vi "VIH Utility - VISRV - Get Datatype Terminal Icon - Ctrl Conatiner.vi"() -> ()   [LabVIEW 2014]
doc: "::: VI Helpeks :::\nCopyright (c) 2000-2026 Konstantin Shifershteyn. All rights reserved."
panel:
  out "Array DAQmx 2":tag[](array[tag])
  in  "Array DAQmx":tag[](array[tag])
  out "DAQmx 2":tag
  in  "DAQmx":tag
  out "Array LV Object 2":refnum<class>[](array[class])
  in  "Array LV Object":refnum<class>[](array[class])
  out "LV Object 2":refnum<class>
  in  "LV Object":refnum<class>
  out "Array Digital Data 2":digitaldata[](array[digital])
  in  "Array Digital Data":digitaldata[](array[digital])
  out "Array Digital Waveform 2":digitalwaveform[](array[waveform])
  in  "Array Digital Waveform":digitalwaveform[](array[waveform])
  out "Array I/O 2":refnum<visa-resource-name>[](array[refnum])
  in  "Array I/O":refnum<visa-resource-name>[](array[refnum])
  out "I/O 2":refnum<visa-resource-name>
  in  "I/O":refnum<visa-resource-name>
  out "Digital Data 2":digitaldata
  out "Digital Waveform 2":digitalwaveform(waveform)={"t0"=timestamp(0 s since 1904-01-01), "dt"=1.0, "Y"={"transitions"=[], "data"=[]}}
  in  "Digital Data":digitaldata
  in  "Digital Waveform":digitalwaveform(waveform)={"t0"=timestamp(0 s since 1904-01-01), "dt"=1.0, "Y"={"transitions"=[], "data"=[]}}
  out "Array WFData 2":dynamicdata[](array[waveform])
  in  "Array WFData":dynamicdata[](array[waveform])
  out "WF Data 2":dynamicdata(waveform)
  in  "WF Data":dynamicdata(waveform)
  out "Array TS 2":timestamp[](array[timestamp])
  in  "Array TS":timestamp[](array[timestamp])
  out "TS 2":timestamp
  in  "TS":timestamp
  out "Array Clust3 2":errorcluster[](array[cluster])
  out "Array Clust2 2":cluster{string}[](array[cluster])
  out "Array Clust1 2":cluster{dbl}[](array[cluster])
  in  "Array Clust3":errorcluster[](array[cluster])
  in  "Array Clust2":cluster{string}[](array[cluster])
  in  "Array Clust1":cluster{dbl}[](array[cluster])
  out "Cluster3 2":errorcluster
  out "Cluster2 2":cluster{string}
  out "Cluster1 2":cluster{dbl}
  in  "Cluster3":errorcluster
  in  "Cluster2":cluster{string}
  in  "Cluster1":cluster{dbl}
  out "Array Enum32 2":enum32{"stub"}[](array[ring])
  out "Array Enum16 2":enum16{"stub"}[](array[ring])
  in  "Array Enum32":enum32{"stub"}[](array[ring])
  in  "Array Enum16":enum16{"stub"}[](array[ring])
  out "Array Enum8 2":enum8{"stub"}[](array[ring])
  in  "Array Enum8":enum8{"stub"}[](array[ring])
  out "Array WF 2":waveform(dbl)[](array[waveform])
  in  "Array WF":waveform(dbl)[](array[waveform])
  out "Array Pict 2":picture[](array[picture])
  in  "Array Pict":picture[](array[picture])
  out "Array Path 2":path[](array[path])
  in  "Array Path":path[](array[path])
  out "Array STR 2":string[](array[string])
  in  "Array STR":string[](array[string])
  out "Array Refnum 2":refnum<vi>[](array[refnum])
  in  "Array Refnum":refnum<vi>[](array[refnum])
  out "Array Bool 2":bool[](array[boolean])
  in  "Array Bool":bool[](array[boolean])
  out "Array CXT 2":cxt[](array[numeric])
  out "Array CDB 2":cdb[](array[numeric])
  out "Array CSG 2":csg[](array[numeric])
  out "Array EXT 2":ext[](array[numeric])
  out "Array DBL 2":dbl[](array[numeric])
  out "Array SGL 2":sgl[](array[numeric])
  out "Array FXP 2":fxp<+/-,8,8>[](array[numeric])
  out "Array U64 2":u64[](array[numeric])
  out "Array U32 2":u32[](array[numeric])
  out "Array U16 2":u16[](array[numeric])
  out "Array U8 2":u8[](array[numeric])
  out "Array I64 2":i64[](array[numeric])
  out "Array I32 2":i32[](array[numeric])
  out "Array I16 2":i16[](array[numeric])
  out "Array I8 2":i8[](array[numeric])
  in  "Array CXT":cxt[](array[numeric])
  in  "Array CDB":cdb[](array[numeric])
  in  "Array CSG":csg[](array[numeric])
  in  "Array EXT":ext[](array[numeric])
  in  "Array DBL":dbl[](array[numeric])
  in  "Array SGL":sgl[](array[numeric])
  in  "Array FXP":fxp<+/-,8,8>[](array[numeric])
  in  "Array U64":u64[](array[numeric])
  in  "Array U32":u32[](array[numeric])
  in  "Array U16":u16[](array[numeric])
  in  "Array U8":u8[](array[numeric])
  in  "Array I64":i64[](array[numeric])
  in  "Array I32":i32[](array[numeric])
  in  "Array I16":i16[](array[numeric])
  in  "Array I8":i8[](array[numeric])
  out "Array VAR 2":variant[](array[variant])
  out "VAR 2":variant
  in  "VAR":variant
  in  "Array VAR":variant[](array[variant])
  out "Waveform 2":waveform(dbl)
  in  "Waveform":waveform(dbl)
  out "Picture 2":picture
  in  "Picture":picture
  out "Enum U32 2":enum32{"stub"}(ring)
  out "Enum U16 2":enum16{"stub"}(ring)
  out "Enum U8 2":enum8{"stub"}(ring)
  in  "Enum U32":enum32{"stub"}(ring)
  in  "Enum U16":enum16{"stub"}(ring)
  in  "Enum U8":enum8{"stub"}(ring)
  out "Path 2":path
  in  "Path":path
  out "Boolean 2":bool
  in  "Boolean":bool
  out "CXT 2":cxt
  out "CDB 2":cdb
  out "CSG 2":csg
  in  "CXT":cxt
  in  "CDB":cdb
  in  "CSG":csg
  out "EXT 2":ext
  out "DBL 2":dbl
  out "SGL 2":sgl
  out "FXP 2":fxp<+,8,8>
  in  "EXT":ext
  in  "DBL":dbl
  in  "SGL":sgl
  in  "FXP":fxp<+,8,8>
  out "Refnum 2":refnum<vi>
  in  "Refnum":refnum<vi>
  out "STR 2":string
  out "U64 2":u64
  out "U32 2":u32
  out "U16 2":u16
  out "U8 2":u8
  out "I64 2":i64
  out "I32 2":i32
  out "I16 2":i16
  out "I8 2":i8
  in  "STR":string
  in  "U64":u64
  in  "U32":u32
  in  "U16":u16
  in  "U8":u8
  in  "I64":i64
  in  "I32":i32
  in  "I16":i16
  in  "I8":i8
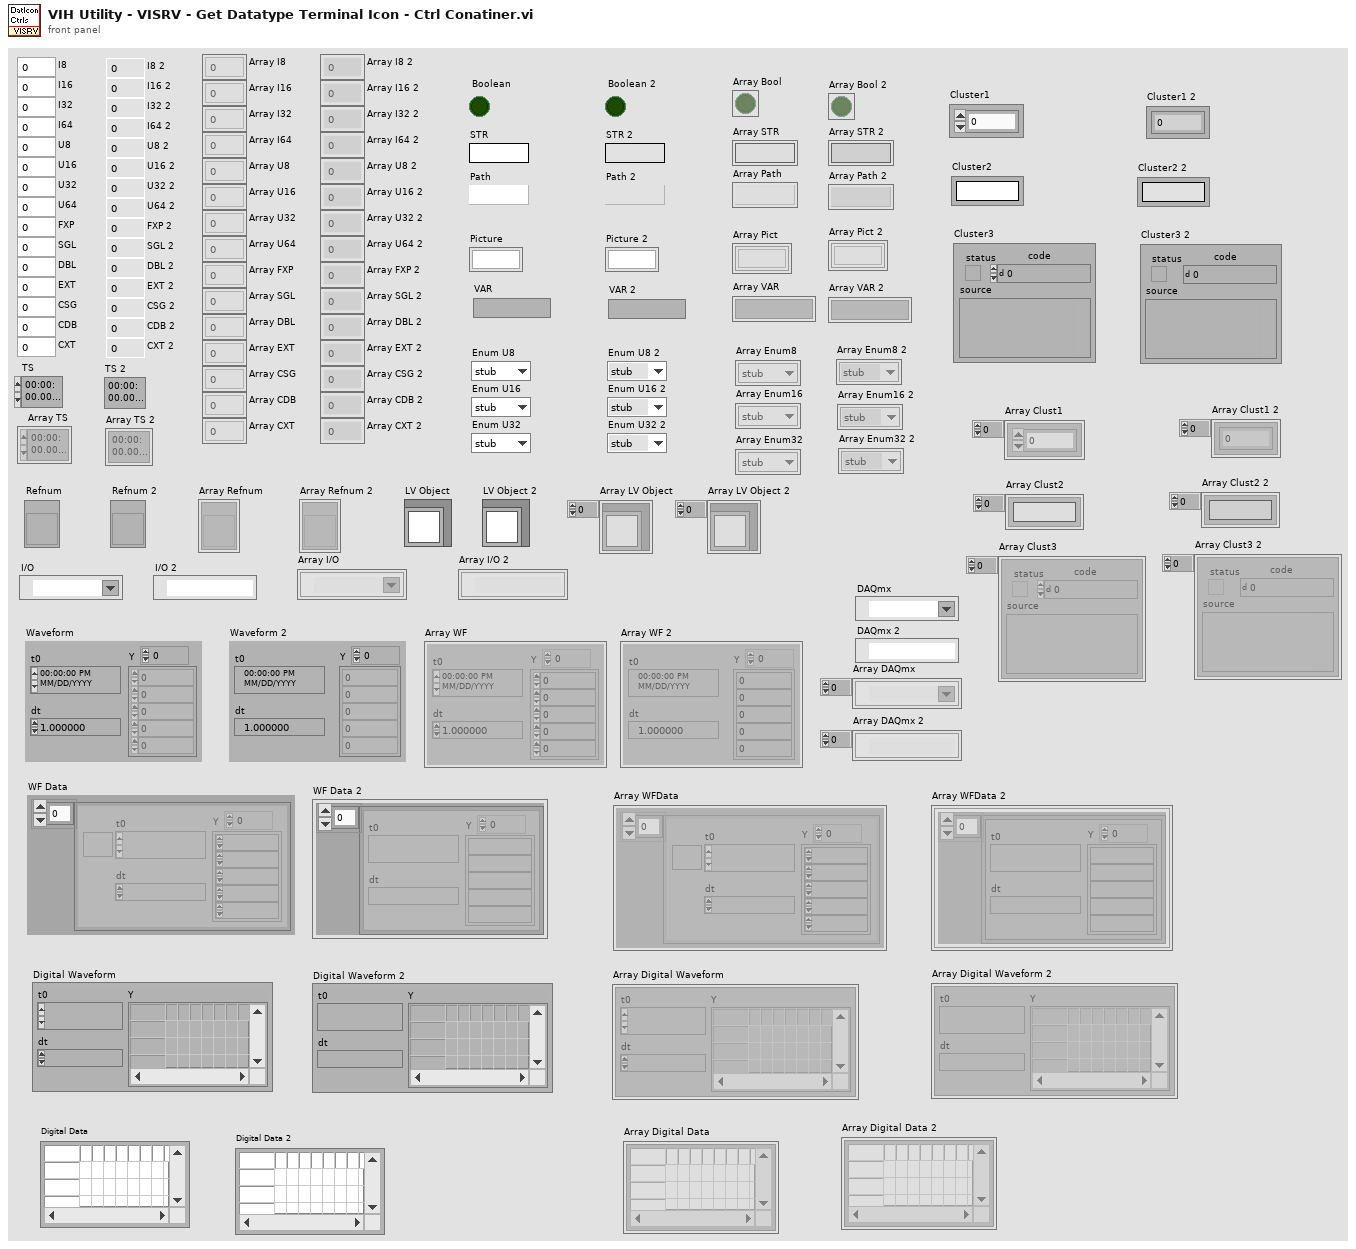
[diagram p1: front panel]
types:
  T1 = enum8{"Enabled", "Disabled", "Disabled and Grayed Out"}
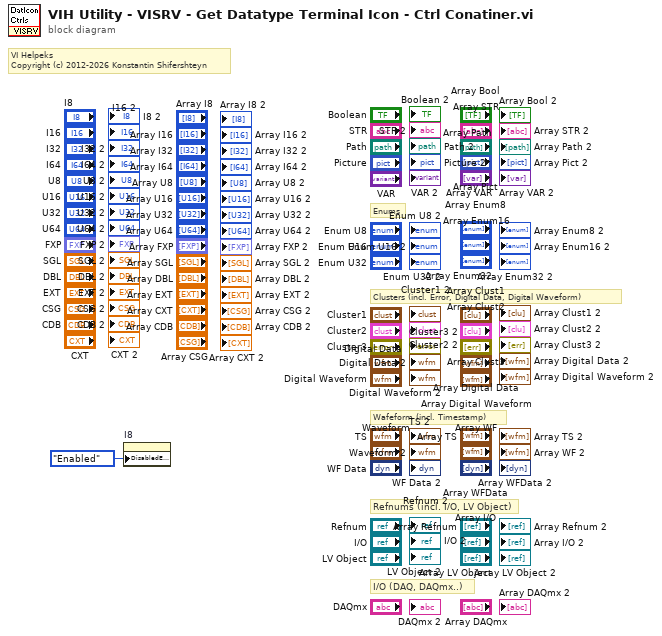
[diagram p0: block diagram]
diagram:
  # "VI Helpeks\nCopyright (c) 2012-2026 Konstantin Shifershteyn"
  # "Enums"
  # "I/O (DAQ, DAQmx..)"
  # "Clusters (incl. Error, Digital Data, Digital Waveform)"
  # "Wafeform (incl. Timestamp)"
  # "Refnums (incl. I/O, LV Object)"
  n1 = property on="I8" class="DigNum (strict)"("DisabledEnum"=T1."Enabled" ("Disabled")) -> ()  [unwired: 2 in, 2 out]
